vi "main.vi"() -> ()   [LabVIEW 2018, in "MediatorPatternDemo.lvclass"]
uses:
  MediatorPatternDemo.lvclass
  User Class/User.lvclass
  ConsoleOut/Print Options.ctl
panel:
  out "error out":errorcluster
  in  "User Name":u16(ring) items=["John", "Robert"]
  in  "Message":string
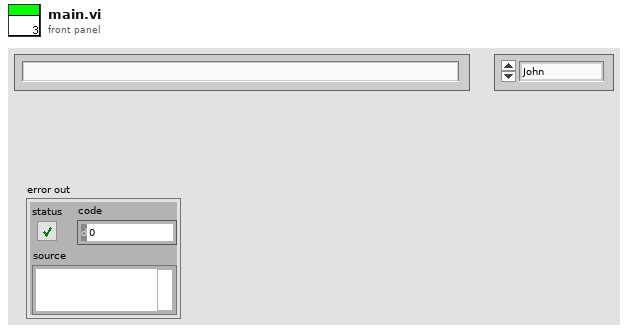
[diagram p1: front panel]
types:
  T1 = typedef "Print Options.ctl" = enum16{"Create", "Get Reference", "Print", "Print Header", "Close"}
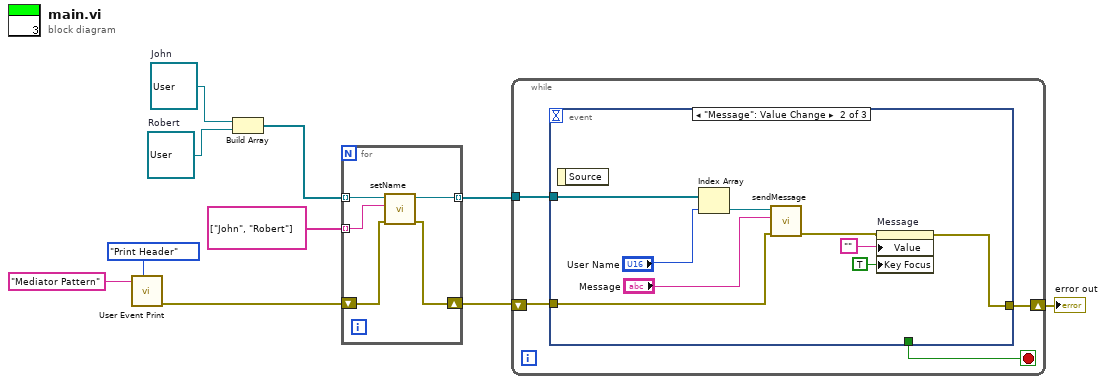
[diagram p0: block diagram]
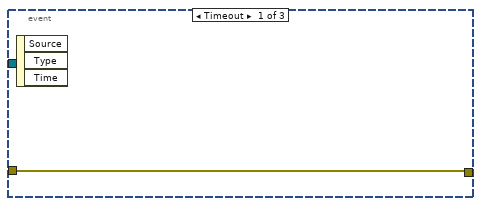
[diagram p2: hidden frame]
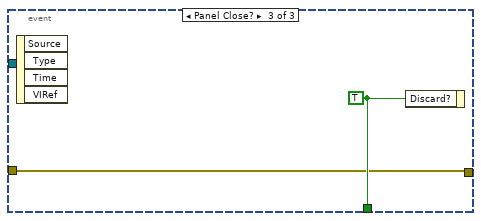
[diagram p3: hidden frame]
diagram:
  w7 = refnum<class "User.lvclass"> refnum  # Robert
  w8 = refnum<class "User.lvclass"> refnum  # John
  n1 = call "User Event Print.vi"("Options"=Print_Options."Print Header", "String to Print"="Mediator Pattern") -> ("error out"=w4:errorcluster)  [unwired: 8 in, 1 out]
  n2 = Build Array(w8, w7) -> (w6:refnum<class "User.lvclass">[])
  n3 = for {
    tunnel: w6 -> [w15] mode=indexing
    tunnel: string[] ["John", "Robert"] ("name") -> [w14] mode=indexing
    tunnel: [w12] -> w3 mode=indexing
    shift-right: [w11] -> w2
    shift-left: w4 -> [w13]
    n4 = call-dynamic "setName.vi"("error in (no error)"=w13, "name"=w14, "User in"=w15) -> ("error out"=w11:errorcluster, "User out"=w12:refnum<class "User.lvclass">)  [unwired: 7 in]
  }
  n5 = while {
    tunnel: w3 -> [w19]
    shift-right: [w16] -> w1
    shift-left: w2 -> [w17]
    stop <- w18 stop-if-true
    n6 = event shown="[1] \"Message\": Value Change" {
      selector: _ -> [_ _ _]
      dyn-events: _ -> [_ _ _]
      timeout: _ -> [_ _ _]
      tunnel: w19 -> [_ w29 _]
      tunnel: [_ _ w31] -> w18
      tunnel: w17 -> [w20 w23 w30]
      tunnel: [w20 w21 w30] -> w16
      event Timeout {
        n7 = event-data() -> ()  [unwired: 1 in, 3 out]
      }
      event "Message": Value Change {
        n8 = event-data() -> ()  [unwired: 1 in, 1 out]
        n9 = Index Array(array=w29, index="User Name") -> (element=w28:refnum<class "User.lvclass">)
        n10 = call-dynamic "sendMessage.vi"("error in (no error)"=w23, "Message"="Message", "User in"=w28) -> ("error out"=w22:errorcluster)  [unwired: 7 in, 1 out]
        n11 = property on="Message" class="Str"(error in=w22, "Value"="", "Key Focus"=TRUE) -> (error out=w21:errorcluster)  [unwired: 1 in, 1 out]
      }
      event Panel Close? {
        w31 = TRUE ("Discard?")
        n12 = event-data() -> ()  [unwired: 1 in, 4 out]
        n13 = event-data("Discard?"=w31) -> ()  [unwired: 1 in, 1 out]
      }
    }
  }
  "error out" <- w1
